vi "Gear_Gate.vi"(0 "MotorControlDevRef":T4={"DeviceStatus"={"status"=FALSE, "code"=0, "source"=""}, "Type"=enum."PWM", "PWM"={"PWM Channel"=enum."Invalid", "DeadBand"={"Name"="", "maxPositivePwm"=0, "minPositivePwm"=0, "centerPwm"=0, "maxNegativePwm"=0, "minNegativePwm"=0, "angularRange"=0}}, "CAN"={"Device Number"=0, "SetOutput VI Ref"=variant(refnum<vi> refnum), "GetOutput VI Ref"=variant(refnum<vi> refnum), "Enable VI Ref"=variant(refnum<vi> refnum), "Disable VI Ref"=variant(refnum<vi> refnum), "Data"=variant}, "Invert"=FALSE}, 1 "Open_Button_Pressed?":bool, 2 "GateParameters":T1={"Scale Positions"={"Forward_StartScale"=0.0, "Reverse_StartScale"=0.0, "Forward_Limit"=0.0, "Reverse_Limit"=0.0}, "Catch_Pos"=1501.0, "Clamp_Pos"=1450.0, "Open_Pos"=1560.0, "Timeout (ms)"=750, "Invert?"=FALSE, "Scale_Factor"=0.1, "Acceptable_Range"=5.0}, 3 "Close_Button_Pressed?":bool, 4 "Potentiometer_Input":dbl=1502.141391720082, 5 "Gate_Pos":T3=enum."Catch") -> (20 "Reached":bool)   [LabVIEW 2016]
uses:
  <vilib>/Rock Robotics/WPI/MotorControl/WPI_MotorControlDeviceRef.ctl
  <vilib>/Rock Robotics/WPI/MotorControl/WPI_MotorControlType.ctl
  <vilib>/Rock Robotics/SystemInterfaces/DIO/FPGA_DIOPWMChannel.ctl
  <vilib>/Rock Robotics/WPI/PWM/WPI_PWMDeadband.ctl
  TypeDefs/GatePos_Type.ctl
  TypeDefs/GateParameters_Type.ctl
  ArgosLib/Miscellaneous/TypeDefs/MotorLimitPositions_Type.ctl
  ArgosLib/ArgosLib.lvlib
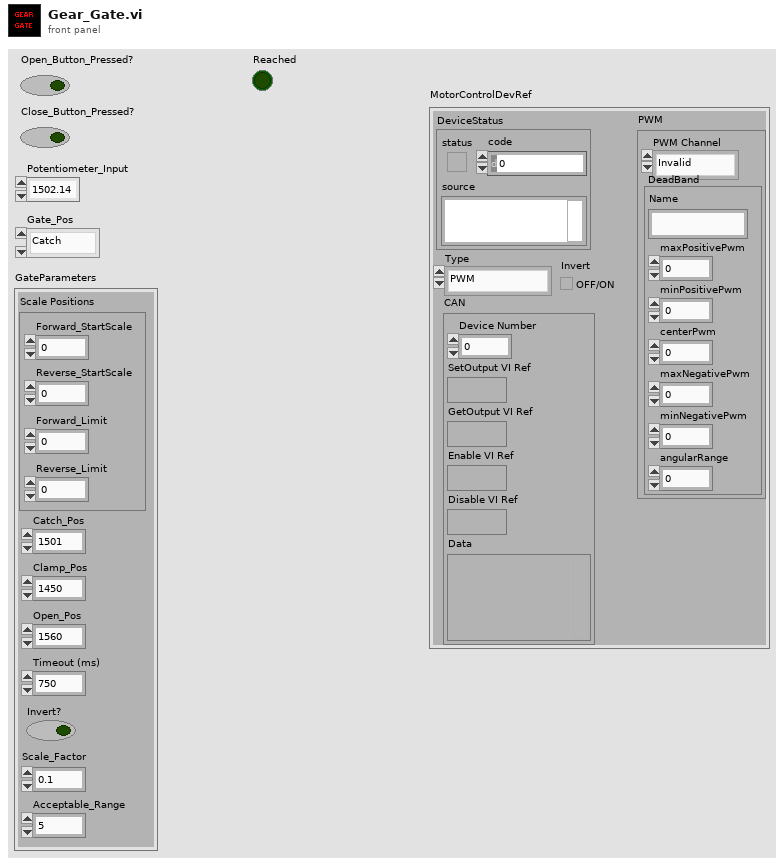
[diagram p1: front panel]
types:
  T1 = typedef "GateParameters_Type.ctl" = cluster{"Scale Positions":T2, "Catch_Pos":dbl, "Clamp_Pos":dbl, "Open_Pos":dbl, "Timeout (ms)":i32, "Invert?":bool, "Scale_Factor":dbl, "Acceptable_Range":dbl}
  T2 = typedef "MotorLimitPositions_Type.ctl" = cluster{"Forward_StartScale":dbl, "Reverse_StartScale":dbl, "Forward_Limit":dbl, "Reverse_Limit":dbl}
  T3 = typedef "GatePos_Type.ctl" = enum16{"Stop", "Catch", "Clamp", "Open"}
  T4 = typedef "WPI_MotorControlDeviceRef.ctl" = cluster{"DeviceStatus":errorcluster, "Type":T5, "PWM":cluster{"PWM Channel":T6, "DeadBand":T7}, "CAN":cluster{"Device Number":u8, "SetOutput VI Ref":variant, "GetOutput VI Ref":variant, "Enable VI Ref":variant, "Disable VI Ref":variant, "Data":variant}, "Invert":bool}
  T5 = typedef "WPI_MotorControlType.ctl" = enum16{"PWM", "CAN"}
  T6 = typedef "FPGA_DIOPWMChannel.ctl" = enum8{"PWM 0", "PWM 1", "PWM 2", "PWM 3", "PWM 4", "PWM 5", "PWM 6", "PWM 7", "PWM 8", "PWM 9", "PWM MXP 0", "PWM MXP 1", "PWM MXP 2", "PWM MXP 3", "PWM MXP 4", "PWM MXP 5", "PWM MXP 6", "PWM MXP 7", "PWM MXP 8", "PWM MXP 9", "Invalid"}
  T7 = typedef "WPI_PWMDeadband.ctl" = cluster{"Name":string, "maxPositivePwm":i32, "minPositivePwm":i32, "centerPwm":i32, "maxNegativePwm":i32, "minNegativePwm":i32, "angularRange":u16}
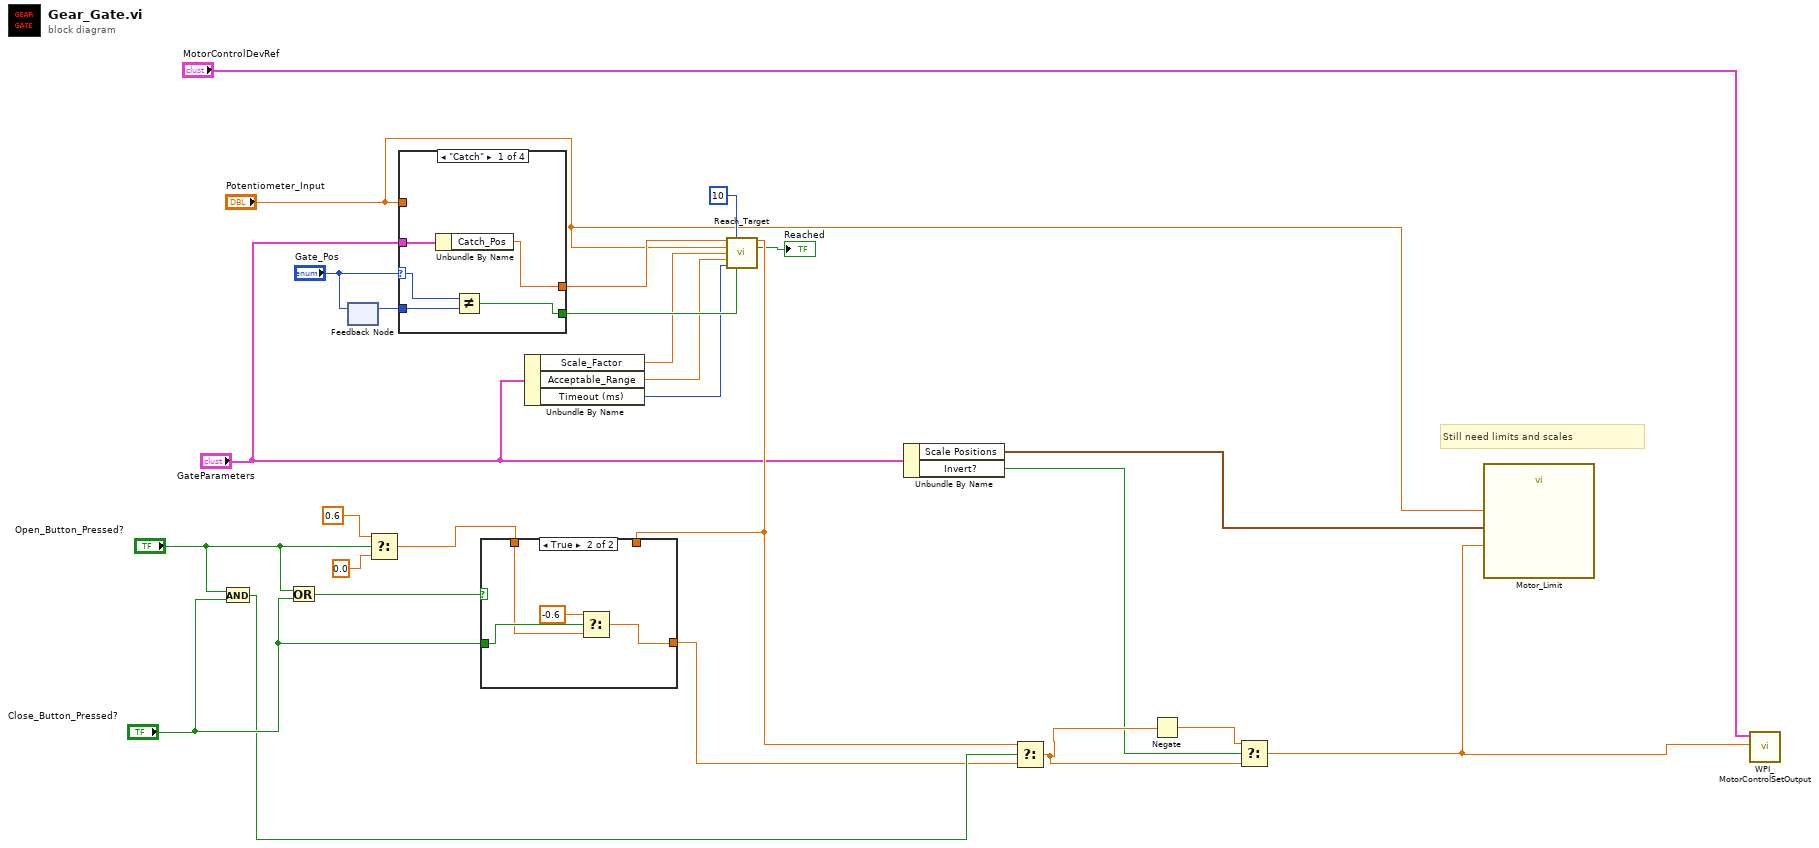
[diagram p0: block diagram]
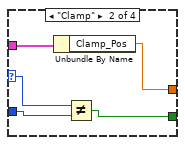
[diagram p3: hidden frame]
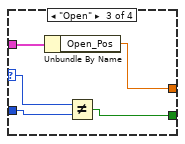
[diagram p4: hidden frame]
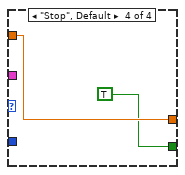
[diagram p5: hidden frame]
diagram:
  # "Still need limits and scales"
  n1 = And(x="Open_Button_Pressed?", y="Close_Button_Pressed?") -> (x .and. y?=w20:bool)
  n2 = Or(x="Open_Button_Pressed?", y="Close_Button_Pressed?") -> (x .or. y?=w21:bool)
  n3 = feedback-in #1("Gate_Pos") -> ()
  n4 = feedback #1() -> (w14:T3)  [unwired: 1 in]
  n5 = Select(t=0.6, s="Open_Button_Pressed?", f=0.0) -> (s? t:f=w19:dbl)
  n6 = case shown="\"Catch\"" "Gate_Pos" {
    selector: "Gate_Pos" -> [w30 w35 w41 _]
    tunnel: [w27 w32 w37 w43] -> w13
    tunnel: "Potentiometer_Input" -> [_ _ _ w43]
    tunnel: [w31 w36 w39 TRUE] -> w16
    tunnel: w14 -> [w29 w34 w40 _]
    tunnel: "GateParameters" -> [w28 w33 w38 _]
    frame "Catch" {
      n7 = Unbundle By Name(w28) -> ("Catch_Pos"=w27:dbl)
      n8 = Not Equal?(x=w30, y=w29) -> (x != y?=w31:bool)
    }
    frame "Clamp" {
      n9 = Unbundle By Name(w33) -> ("Clamp_Pos"=w32:dbl)
      n10 = Not Equal?(x=w35, y=w34) -> (x != y?=w36:bool)
    }
    frame "Open" {
      n11 = Unbundle By Name(w38) -> ("Open_Pos"=w37:dbl)
      n12 = Not Equal?(x=w41, y=w40) -> (x != y?=w39:bool)
    }
    frame "Stop", Default {
    }
  }
  n13 = Unbundle By Name("GateParameters") -> ("Scale_Factor"=w6:dbl, "Acceptable_Range"=w5:dbl, "Timeout (ms)"=w4:i32)
  n14 = call "Reach_Target.vi"("Target_Position"=w13, "Maintain_Samples"=10 ("Num samples"), "Current_Position"="Potentiometer_Input", "Scale_Factor"=w6, "Acceptable_Range"=w5, "Timeout (ms)"=w4, "Reset"=w16) -> ("Motor_Value"=w11:dbl, "Reached"=→"Reached":bool)  [unwired: 7 in]
  n15 = case shown="True" w21 {
    tunnel: [w44 w48] -> w18
    tunnel: "Close_Button_Pressed?" -> [_ w47]
    tunnel: w19 -> [_ w46]
    tunnel: w11 -> [w44 _]
    frame False {
    }
    frame True {
      n16 = Select(t=-0.6, s=w47, f=w46) -> (s? t:f=w48:dbl)
    }
  }
  n17 = Unbundle By Name("GateParameters") -> ("Scale Positions"=w1:T2, "Invert?"=w2:bool)
  n18 = Select(t=w11, s=w20, f=w18) -> (s? t:f=w7:dbl)
  n19 = Negate(x=w7) -> (-x=w8:dbl)
  n20 = Select(t=w8, s=w2, f=w7) -> (s? t:f=w9:dbl)
  n21 = call "Motor_Limit.vi"("Current_Pos"="Potentiometer_Input", "Motor_Speed"=w9, "Scale Positions"=w1) -> ()  [unwired: 15 in, 2 out]
  n22 = call <vilib>:"WPI_MotorControlSetOutput.vi"("Output"=w9, "MotorControlDevRef"="MotorControlDevRef") -> ()  [unwired: 7 in, 3 out]
